vi "Teleop.vi"(10 "Match Info":T1={"Autonomous Elapsed Seconds"=0.0, "TeleOp Elapsed Seconds"=192.47, "Disabled Elapsed Seconds"=11.36, "Visited Autonomous"=FALSE, "Visited TeleOp"=TRUE, "Visited Disabled"=TRUE, "Autonomous Settings"={"Autonomous Style"=enum."Independent", "VI Refnum"=refnum}}, 11 "Call Context":T2=enum."Stop") -> ()   [LabVIEW 2015]
doc: "This VI is called for each TeleOp packet received from the DS where the robot is not disabled. It is often used to read from the joysticks and update I/O or to update setpoints for timed control loops. It should complete and return within 20 milliseconds or it may miss DS packets."
uses:
  <vilib>/Rock Robotics/WPI/DriverStation/WPI_DriverStationDerivedRobotMode.ctl
  <vilib>/Rock Robotics/WPI/DriverStation/WPI_DriverStationMatch Info.ctl
  <vilib>/Rock Robotics/WPI/Solenoid/WPI_SolenoidValue.ctl
  <vilib>/Rock Robotics/WPI/Utilities/WPI_GetSetVariantRefNum.vi
  <vilib>/Rock Robotics/Network Tables/NT Write Numeric Array.vi
  <vilib>/Rock Robotics/WPI/Solenoid/WPI_SolenoidSetEnum.vi
  Robot Global Data.vi
panel:
  in  "Only 1 player":bool
  in  "Controller 2 Upper Limit":dbl=0.4999999999999996 min=0.0 max=1.0 step=0.05 format="%#_13g"
  in  "Angle X":i32=25 min=0 max=170 step=5
  in  "Angle Y":i32=170 min=0 max=170 step=5
  in  "Delta servo caméra":u16=5
  in  "Forza style":bool=TRUE
  in  "Toggle cheval":i32=2 min=0 max=9 step=1
  in  "Toggle Lanceur":i32=3 min=0 max=9 step=1
  in  "Take button":i32=5 min=0 max=9 step=1
  in  "Shoot button":i32=4 min=0 max=9 step=1
  in  "Stop button":i32=1 min=0 max=9 step=1
  in  "Take Speed":dbl=0.49999999999999994 min=0.0 max=1.0 step=0.05 format="%#_13g"
  in  "Shoot Speed":dbl=0.9 min=0.0 max=1.0 step=0.05
  # "Lanceur"
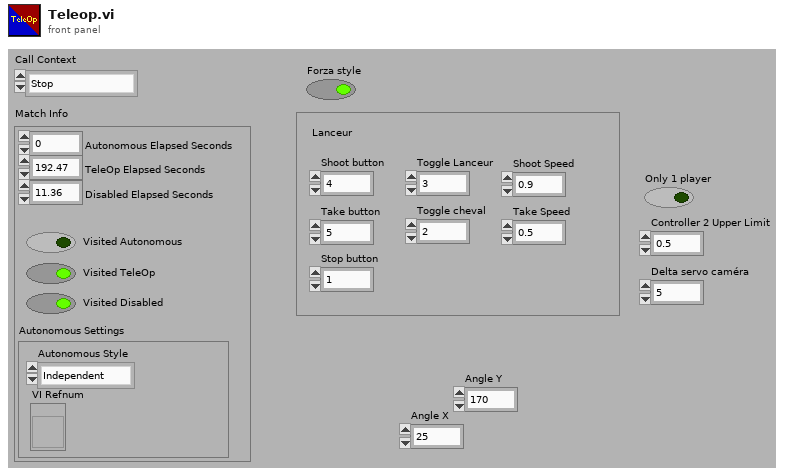
[diagram p1: front panel]
types:
  T1 = typedef "WPI_DriverStationMatch Info.ctl" = cluster{"Autonomous Elapsed Seconds":dbl, "TeleOp Elapsed Seconds":dbl, "Disabled Elapsed Seconds":dbl, "Visited Autonomous":bool, "Visited TeleOp":bool, "Visited Disabled":bool, "Autonomous Settings":cluster{"Autonomous Style":enum16{"Iterative", "Independent"}, "VI Refnum":refnum<vi>}}
  T2 = typedef "WPI_DriverStationDerivedRobotMode.ctl" = enum16{"Init", "Execute", "Stop"}
  T3 = typedef "WPI_SolenoidValue.ctl" = enum16{"Off", "On", "Forward", "Reverse"}
  T4 = typedef "WPI_JoystickDevRef.ctl" = cluster{"Device":T5}
  T5 = typedef "WPI_JoystickDeviceEnum.ctl" = enum16{"USB 0", "USB 1", "USB 2", "USB 3", "USB 4", "USB 5"}
  T6 = cluster{"Axes[0]":dbl, "Axes[1]":dbl, "Axes[2]":dbl, "Axes[3]":dbl, "Axes[4]":dbl, "Axes[5]":dbl, "Axes[6]":dbl, "Axes[7]":dbl, "Axes[8]":dbl}
  T7 = typedef "WPI_ServoDeviceRef.ctl" = cluster{"DeviceStatus":errorcluster, "PWM Channel":T8, "DeadBand":T9}
  T8 = typedef "FPGA_DIOPWMChannel.ctl" = enum8{"PWM 0", "PWM 1", "PWM 2", "PWM 3", "PWM 4", "PWM 5", "PWM 6", "PWM 7", "PWM 8", "PWM 9", "PWM MXP 0", "PWM MXP 1", "PWM MXP 2", "PWM MXP 3", "PWM MXP 4", "PWM MXP 5", "PWM MXP 6", "PWM MXP 7", "PWM MXP 8", "PWM MXP 9", "Invalid"}
  T9 = typedef "WPI_PWMDeadband.ctl" = cluster{"Name":string, "maxPositivePwm":i32, "minPositivePwm":i32, "centerPwm":i32, "maxNegativePwm":i32, "minNegativePwm":i32, "angularRange":u16}
  T10 = typedef "WPI_RobotDriveDevRef.ctl" = cluster{"DevStatus":errorcluster, "Motors[]":T11[], "Square Inputs":bool, "Max Output":dbl}
  T11 = typedef "WPI_MotorControlDeviceRef.ctl" = cluster{"DeviceStatus":errorcluster, "Type":T12, "PWM":cluster{"PWM Channel":T8, "DeadBand":T9}, "CAN":cluster{"Device Number":u8, "Control Mode":T13, "Semaphore":T14, "Max Vout":dbl, "TalonSRX Control Mode":T15}, "Invert":bool}
  T12 = typedef "WPI_MotorControlType.ctl" = enum16{"PWM", "CAN", "CANTalonSRX"}
  T13 = typedef "WPI_CANJaguar_ControlMode.ctl" = enum8{"Percent VBus", "Current", "Speed", "Position", "Voltage"}
  T14 = typedef "Semaphore RefNum" = refnum<k1>
  T15 = typedef "WPI_CANTalonSRX_APIControlMode.ctl" = enum8{"Percent VBus", "Speed", "Position", "Slave", "Unchanged / Invalid", "Voltage Compensation", "Current", "Motion Profile"}
  T16 = typedef "WPI_SolenoidDevRef.ctl" = cluster{"DevStatus":errorcluster, "Pneumatics Control Module":u8, "Forward Solenoid Channel":T17, "Reverse Solenoid Channel":T17}
  T17 = typedef "WPI_SolenoidChannel.ctl" = enum8{"Solenoid 0", "Solenoid 1", "Solenoid 2", "Solenoid 3", "Solenoid 4", "Solenoid 5", "Solenoid 6", "Solenoid 7", "Invalid"}
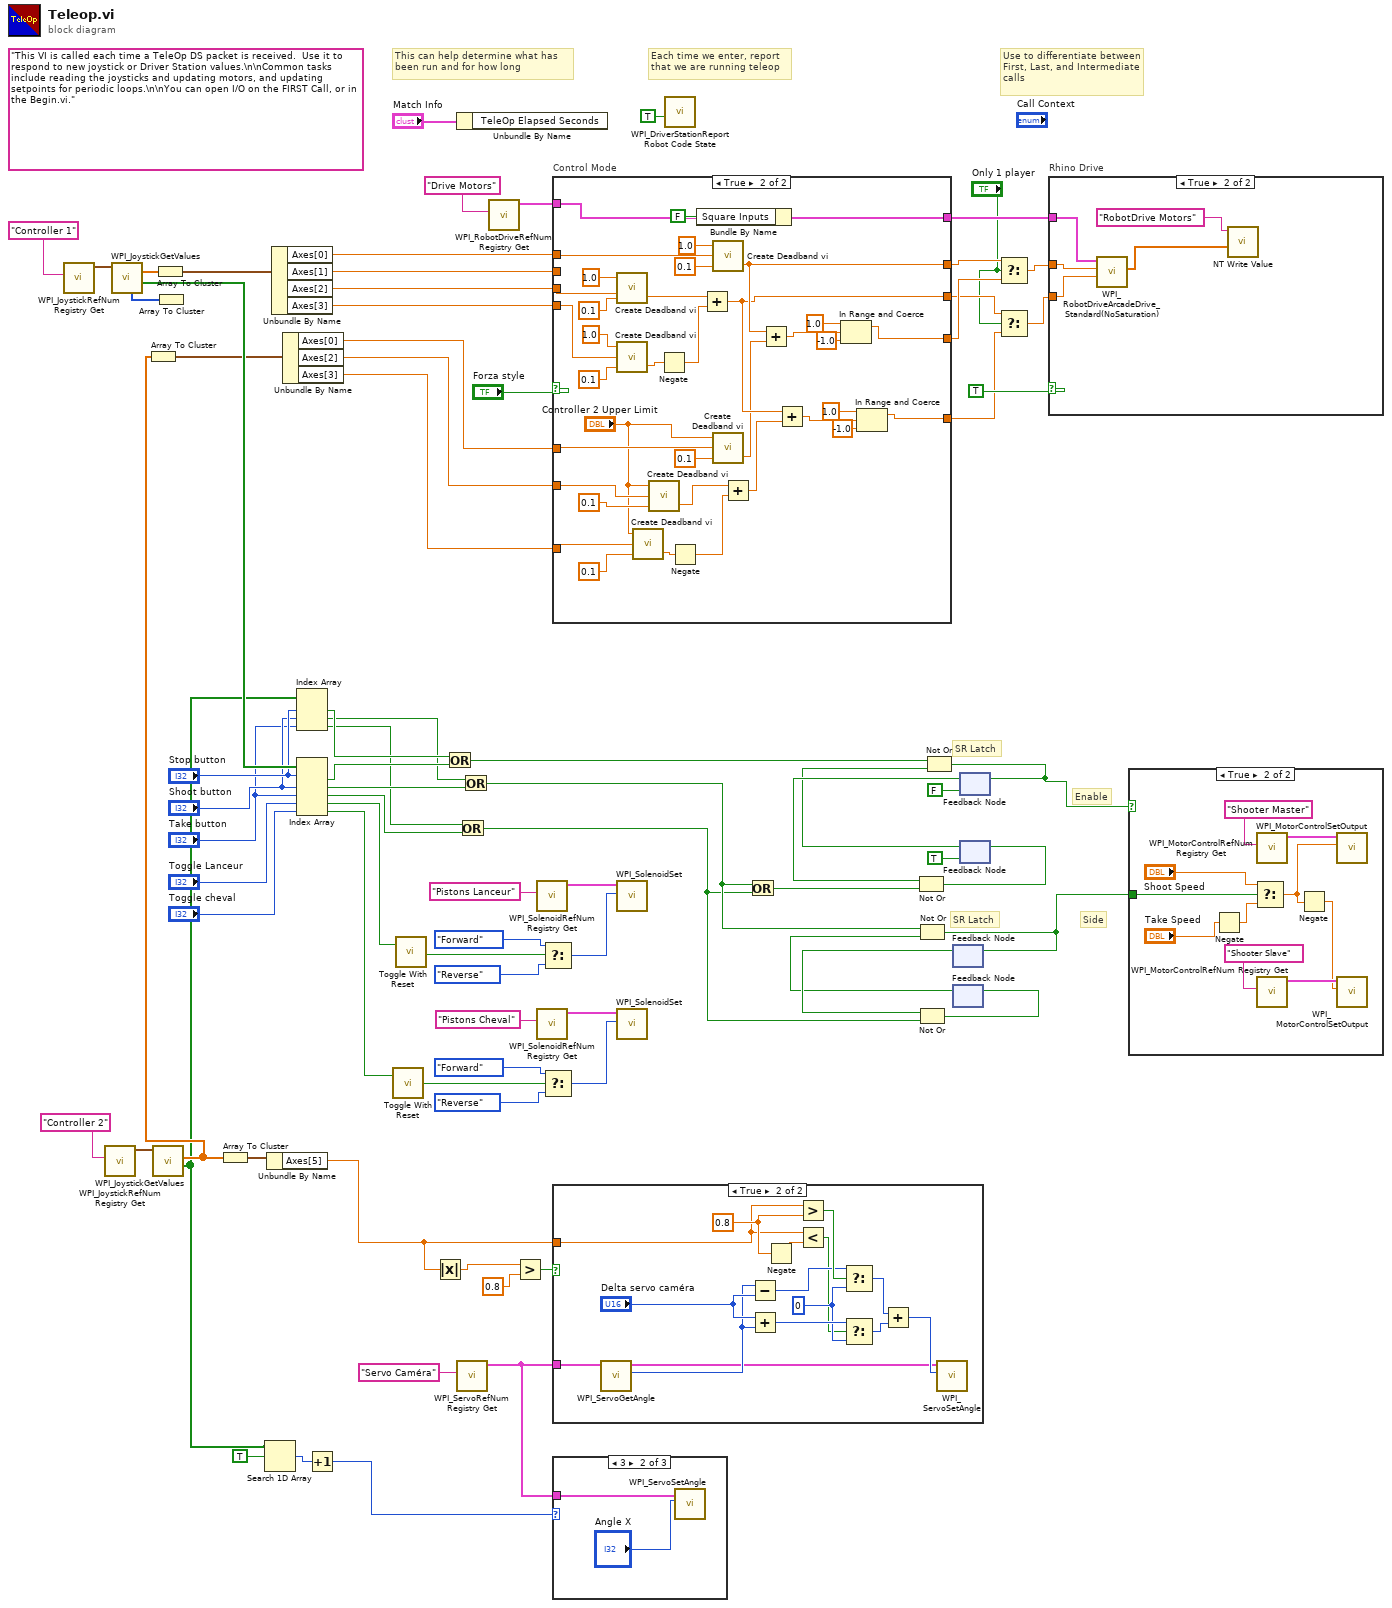
[diagram p0: block diagram]
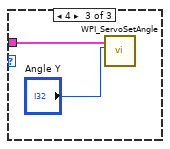
[diagram p3: hidden frame]
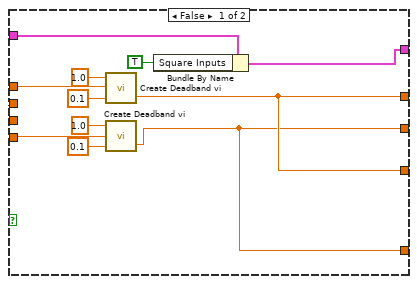
[diagram p5: hidden frame]
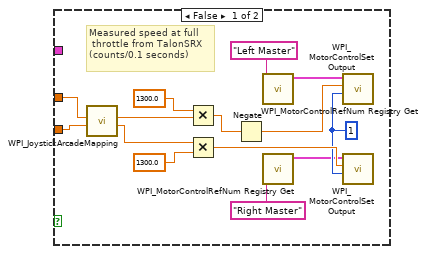
[diagram p6: hidden frame]
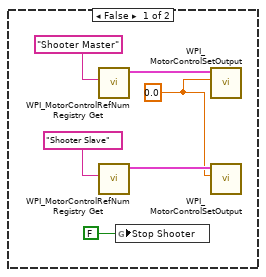
[diagram p7: hidden frame]
diagram:
  (unwired) "This VI is called each time a TeleOp DS packet is received.  Use it to respond to new joystick or Driver Station values.\n\nCommon tasks include reading the joysticks and updating motors, and updating setpoints for periodic loops.\n\nYou can open I/O on the FIRST Call, or in the Begin.vi."
  # "Side"
  # "Enable"
  # "SR Latch"
  # "SR Latch"
  # "Each time we enter, report that we are running teleop"
  # "Use to differentiate between First, Last, and Intermediate calls"
  # "This can help determine what has\nbeen run and for how long"
  n1 = call <vilib>:"WPI_JoystickRefNum Registry Get.vi"("refnum name"="Controller 1") -> ("JoystickDevRef"=w79:T4)  [unwired: 1 in, 9 out]
  n2 = call <vilib>:"WPI_JoystickRefNum Registry Get.vi"("refnum name"="Controller 2") -> ("JoystickDevRef"=w46:T4)  [unwired: 1 in, 9 out]
  n3 = call <vilib>:"WPI_JoystickGetValues.vi"("JoystickDevRef"=w79) -> ("Buttons"=w48:bool[], "Axes"=w49:dbl[], "POVs"=w47:i16[])  [unwired: 6 in, 2 out]
  n4 = call <vilib>:"WPI_JoystickGetValues.vi"("JoystickDevRef"=w46) -> ("Buttons"=w12:bool[], "Axes"=w23:dbl[])  [unwired: 6 in, 3 out]
  n5 = Array To Cluster(array=w23) -> (cluster=w24:T6)
  n6 = Array To Cluster(array=w49) -> (cluster=w77:T6)
  n7 = Array To Cluster(array=w47) -> ()  [unwired: 1 out]
  n8 = Array To Cluster(array=w23) -> (cluster=w32:T6)
  n9 = Search 1D Array(1D array=w12, element=TRUE) -> (index of element=w26:i32)  [unwired: 1 in]
  n10 = Unbundle By Name(w32) -> ("Axes[5]"=w31:dbl)
  n11 = Unbundle By Name(w77) -> ("Axes[0]"=w41:dbl, "Axes[1]"=w40:dbl, "Axes[2]"=w43:dbl, "Axes[3]"=w42:dbl)
  n12 = Unbundle By Name(w24) -> ("Axes[0]"=w22:dbl, "Axes[2]"=w21:dbl, "Axes[3]"=w20:dbl)
  n13 = Index Array(array=w12, index #1="Stop button", index #2="Shoot button", index #3="Take button") -> (element #1=w6:bool, element #2=w4:bool, element #3=w1:bool)
  n14 = Index Array(array=w48, index #1="Stop button", index #2="Shoot button", index #3="Take button", index #4="Toggle Lanceur", index #5="Toggle cheval") -> (element #1=w7:bool, element #2=w66:bool, element #3=w3:bool, element #4=w62:bool, element #5=w61:bool)
  n15 = Increment(x=w26) -> (x+1=w25:i32)
  n16 = call "Toggle With Reset.vi"("Boolean"=w61) -> ("Driver Switch 2"=w44:bool)  [unwired: 1 in]
  n17 = call "Toggle With Reset.vi"("Boolean"=w62) -> ("Driver Switch 2"=w50:bool)  [unwired: 1 in]
  n18 = Absolute Value(x=w31) -> (abs(x)=w29:dbl)
  n19 = Or(x=w6, y=w7) -> (x .or. y?=w8:bool)
  n20 = Unbundle By Name("Match Info") -> ()  [unwired: 1 out]
  n21 = call <vilib>:"WPI_ServoRefNum Registry Get.vi"("refnum name"="Servo Caméra") -> ("ServoDeviceRef"=w33:T7)  [unwired: 9 in, 1 out]
  n22 = Or(x=w1, y=w3) -> (x .or. y?=w2:bool)
  n23 = Or(x=w4, y=w66) -> (x .or. y?=w5:bool)
  n24 = call <vilib>:"WPI_RobotDriveRefNum Registry Get.vi"("refnum name"="Drive Motors") -> ("RobotDriveDevRef"=w36:T10)  [unwired: 1 in, 9 out]
  n25 = Greater?(x=w29, y=0.8) -> (0:w30:bool)
  n26 = call <vilib>:"WPI_SolenoidRefNum Registry Get.vi"("refnum name"="Pistons Lanceur") -> ("SolenoidDevRef"=w58:T16)  [unwired: 9 in, 1 out]
  n27 = call <vilib>:"WPI_SolenoidRefNum Registry Get.vi"("refnum name"="Pistons Cheval") -> ("SolenoidDevRef"=w54:T16)  [unwired: 9 in, 1 out]
  n28 = Select(t=WPI_SolenoidValue."Forward" ("Value"), s=w50, f=WPI_SolenoidValue."Reverse" ("Value")) -> (s? t:f=w60:T3)
  n29 = Select(t=WPI_SolenoidValue."Forward" ("Value"), s=w44, f=WPI_SolenoidValue."Reverse" ("Value")) -> (s? t:f=w52:T3)
  n30 = case "Control Mode" shown="True" "Forza style" {
    tunnel: w43 -> [_ w121]
    tunnel: w42 -> [_ w120]
    tunnel: w41 -> [w89 w122]
    tunnel: w40 -> [w88 _]
    tunnel: [w83 w104] -> w19
    tunnel: [w82 w103] -> w14
    tunnel: [w90 w115] -> w38
    tunnel: w36 -> [w91 w115]
    tunnel: w22 -> [_ w108]
    tunnel: w21 -> [_ w106]
    tunnel: w20 -> [_ w107]
    tunnel: [w83 w99] -> w18
    tunnel: [w82 w93] -> w15
    frame False {
      n31 = call "Create Deadband vi.vi"("Input Deadband"=0.1, "Input"=w89, "Output Upper Limit"=1.0) -> ("Output"=w83:dbl)  [unwired: 1 in]
      n32 = call "Create Deadband vi.vi"("Input Deadband"=0.1, "Input"=w88, "Output Upper Limit"=1.0) -> ("Output"=w82:dbl)  [unwired: 1 in]
      n33 = Bundle By Name(cluster=w91, "Square Inputs"=TRUE) -> (w90:T10)
    }
    frame True {
      n34 = call "Create Deadband vi.vi"("Input Deadband"=0.1, "Input"=w121, "Output Upper Limit"=1.0) -> ("Output"=w125:dbl)  [unwired: 1 in]
      n35 = call "Create Deadband vi.vi"("Input Deadband"=0.1, "Input"=w120, "Output Upper Limit"=1.0) -> ("Output"=w128:dbl)  [unwired: 1 in]
      n36 = call "Create Deadband vi.vi"("Input Deadband"=0.1, "Input"=w107, "Output Upper Limit"="Controller 2 Upper Limit") -> ("Output"=w109:dbl)  [unwired: 1 in]
      n37 = call "Create Deadband vi.vi"("Input Deadband"=0.1, "Input"=w106, "Output Upper Limit"="Controller 2 Upper Limit") -> ("Output"=w111:dbl)  [unwired: 1 in]
      n38 = Negate(x=w128) -> (-x=w119:dbl)
      n39 = Negate(x=w109) -> (-x=w113:dbl)
      n40 = Bundle By Name(cluster=w115, "Square Inputs"=FALSE) -> ()  [unwired: 1 out]
      n41 = Add(x=w125, y=w119) -> (x+y=w103:dbl)
      n42 = call "Create Deadband vi.vi"("Input Deadband"=0.1, "Input"=w122, "Output Upper Limit"=1.0) -> ("Output"=w104:dbl)  [unwired: 1 in]
      n43 = call "Create Deadband vi.vi"("Input Deadband"=0.1, "Input"=w108, "Output Upper Limit"="Controller 2 Upper Limit") -> ("Output"=w102:dbl)  [unwired: 1 in]
      n44 = Add(x=w111, y=w113) -> (x+y=w101:dbl)
      n45 = Add(x=w104, y=w102) -> (x+y=w100:dbl)
      n46 = Add(x=w103, y=w101) -> (x+y=w96:dbl)
      n47 = In Range and Coerce(upper limit=1.0, x=w100, lower limit=-1.0) -> (coerced(x)=w99:dbl)  [unwired: 1 out]
      n48 = In Range and Coerce(upper limit=1.0, x=w96, lower limit=-1.0) -> (coerced(x)=w93:dbl)  [unwired: 1 out]
    }
  }
  n49 = case shown="True" w30 {
    tunnel: w33 -> [_ w129]
    tunnel: w31 -> [_ w133]
    frame False {
    }
    frame True {
      w135 = 0.8 ("y")
      w140 = u16 0 ("f")
      n50 = call <vilib>:"WPI_ServoGetAngle.vi"("ServoDeviceRef"=w129) -> ("ServoDeviceRef"=w130:T7, "Angle"=w131:u16)  [unwired: 7 in, 1 out]
      n51 = Subtract(x=w131, y="Delta servo caméra") -> (x-y=w141:u16)
      n52 = Add(x="Delta servo caméra", y=w131) -> (x+y=w142:u16)
      n53 = Negate(x=w135) -> (-x=w134:dbl)
      n54 = Greater?(x=w133, y=w135) -> (0:w143:bool)
      n55 = Less?(x=w133, y=w134) -> (x < y?=w139:bool)
      n56 = Select(t=w141, s=w143, f=w140) -> (s? t:f=w138:u16)
      n57 = Select(t=w142, s=w139, f=w140) -> (s? t:f=w137:u16)
      n58 = Add(x=w138, y=w137) -> (x+y=w136:u16)
      n59 = call <vilib>:"WPI_ServoSetAngle.vi"("Angle"=w136, "ServoDeviceRef"=w130) -> ()  [unwired: 8 in, 2 out]
    }
  }
  n60 = case shown="3" w25 {
    tunnel: w33 -> [_ w144 w147]
    frame 0, Default {
      # "Rien"
    }
    frame 3 {
      n61 = call <vilib>:"WPI_ServoSetAngle.vi"("Angle"="Angle X", "ServoDeviceRef"=w144) -> ()  [unwired: 8 in, 2 out]
    }
    frame 4 {
      n62 = call <vilib>:"WPI_ServoSetAngle.vi"("Angle"="Angle Y", "ServoDeviceRef"=w147) -> ()  [unwired: 8 in, 2 out]
    }
  }
  n63 = call-poly <vilib>:"WPI_SolenoidSet.vi"("Value"=w60, "SolenoidDevRef"=w58) -> ()  [unwired: 8 in, 2 out]
  n64 = call-poly <vilib>:"WPI_SolenoidSet.vi"("Value"=w52, "SolenoidDevRef"=w54) -> ()  [unwired: 8 in, 2 out]
  n65 = call <vilib>:"WPI_DriverStationReport Robot Code State.vi"("TeleOp"=TRUE ("Autonomous")) -> ()  [unwired: 10 in, 1 out]
  n66 = Or(x=w5, y=w2) -> (x .or. y?=w69:bool)
  n67 = feedback #1() -> (w76:bool)  [unwired: 1 in]
  n68 = Not Or(1:w2, 2:w76) -> (0:w75:bool)
  n69 = feedback #2() -> (w74:bool)  [unwired: 1 in]
  n70 = Not Or(1:w74, 2:w5) -> (0:w73:bool)
  n71 = feedback-in #1(w73) -> ()
  n72 = feedback-in #2(w75) -> ()
  n73 = feedback #3(FALSE) -> (w72:bool)
  n74 = Not Or(1:w69, 2:w72) -> (0:w71:bool)
  n75 = feedback #4(TRUE) -> (w70:bool)
  n76 = Not Or(1:w70, 2:w8) -> (0:w63:bool)
  n77 = feedback-in #3(w63) -> ()
  n78 = feedback-in #4(w71) -> ()
  n79 = Select(t=w19, s="Only 1 player", f=w18) -> (s? t:f=w17:dbl)
  n80 = Select(t=w14, s="Only 1 player", f=w15) -> (s? t:f=w16:dbl)
  n81 = case "Rhino Drive" shown="True" TRUE {
    tunnel: w17 -> [w149 w165]
    tunnel: w16 -> [w148 w164]
    tunnel: w38 -> [_ w166]
    frame False {
      w156 = u8 1 ("Sync Group / Parameter Slot")
      # "Measured speed at full\n throttle from TalonSRX\n(counts/0.1 seconds)"
      n82 = call <vilib>:"WPI_JoystickArcadeMapping.vi"("Y axis value"=w148, "X axis value"=w149) -> ("Right Motor Value"=w151:dbl, "Left Motor Value"=w150:dbl)  [unwired: 8 in]
      n83 = Multiply(x=1300.0, y=w150) -> (x*y=w157:dbl)
      n84 = Multiply(x=w151, y=1300.0) -> (x*y=w159:dbl)
      n85 = Negate(x=w157) -> (-x=w158:dbl)
      n86 = call <vilib>:"WPI_MotorControlRefNum Registry Get.vi"("refnum name"="Left Master") -> ("MotorControlDevRef"=w154:T11)  [unwired: 9 in, 1 out]
      n87 = call <vilib>:"WPI_MotorControlRefNum Registry Get.vi"("refnum name"="Right Master") -> ("MotorControlDevRef"=w155:T11)  [unwired: 9 in, 1 out]
      n88 = call <vilib>:"WPI_MotorControlSetOutput.vi"("Sync Group / Parameter Slot"=w156, "Output"=w158, "MotorControlDevRef"=w154) -> ()  [unwired: 6 in, 3 out]
      n89 = call <vilib>:"WPI_MotorControlSetOutput.vi"("Sync Group / Parameter Slot"=w156, "Output"=w159, "MotorControlDevRef"=w155) -> ()  [unwired: 6 in, 3 out]
    }
    frame True {
      n90 = call <vilib>:"WPI_RobotDriveArcadeDrive_Standard(NoSaturation).vi"("Y axis value"=w164, "X axis value"=w165, "RobotDriveDevRef"=w166) -> ("Motor Values"=w162:dbl[])  [unwired: 1 in, 7 out]
      n91 = call-poly <vilib>:"NT Write Value.vi"("Numeric Array"=w162, "Name"="RobotDrive Motors") -> ()  [unwired: 9 in, 1 out]
    }
  }
  n92 = case shown="True" w63 {
    tunnel: w73 -> [_ w180]
    frame False {
      w168 = 0.0 ("Output")
      n93 = call <vilib>:"WPI_MotorControlRefNum Registry Get.vi"("refnum name"="Shooter Master") -> ("MotorControlDevRef"=w172:T11)  [unwired: 9 in, 1 out]
      n94 = call <vilib>:"WPI_MotorControlRefNum Registry Get.vi"("refnum name"="Shooter Slave") -> ("MotorControlDevRef"=w169:T11)  [unwired: 9 in, 1 out]
      n95 = global write "Robot Global Data.vi" "Stop Shooter"(FALSE ("Shooter Stop")) -> ()
      n96 = call <vilib>:"WPI_MotorControlSetOutput.vi"("Output"=w168, "MotorControlDevRef"=w172) -> ()  [unwired: 7 in, 3 out]
      n97 = call <vilib>:"WPI_MotorControlSetOutput.vi"("Output"=w168, "MotorControlDevRef"=w169) -> ()  [unwired: 7 in, 3 out]
    }
    frame True {
      n98 = Negate(x="Take Speed") -> (-x=w177:dbl)
      n99 = Select(t="Shoot Speed", s=w180, f=w177) -> (s? t:f=w175:dbl)
      n100 = call <vilib>:"WPI_MotorControlRefNum Registry Get.vi"("refnum name"="Shooter Master") -> ("MotorControlDevRef"=w181:T11)  [unwired: 9 in, 1 out]
      n101 = call <vilib>:"WPI_MotorControlRefNum Registry Get.vi"("refnum name"="Shooter Slave") -> ("MotorControlDevRef"=w176:T11)  [unwired: 9 in, 1 out]
      n102 = Negate(x=w175) -> (-x=w173:dbl)
      n103 = call <vilib>:"WPI_MotorControlSetOutput.vi"("Output"=w175, "MotorControlDevRef"=w181) -> ()  [unwired: 7 in, 3 out]
      n104 = call <vilib>:"WPI_MotorControlSetOutput.vi"("Output"=w173, "MotorControlDevRef"=w176) -> ()  [unwired: 7 in, 3 out]
    }
  }
